vi "VI control.vi"() -> ()   [LabVIEW 2021]
uses:
  <vilib>/DAQmx/read.llb/DAQmx Read (Counter DBL 1Chan 1Samp).vi
  <vilib>/DAQmx/write.llb/DAQmx Write (Analog DBL 1Chan 1Samp).vi
  <vilib>/DAQmx/write.llb/DAQmx Write (Digital 1D Bool 1Chan 1Samp).vi
  <vilib>/DAQmx/create/channels.llb/DAQmx Create Channel (CI-Position-Angular Encoder).vi
  <vilib>/DAQmx/create/channels.llb/DAQmx Create Channel (AO-Voltage-Basic).vi
  <vilib>/DAQmx/create/channels.llb/DAQmx Create Channel (DO-Digital Output).vi
  <vilib>/DAQmx/miscellaneous.llb/DAQmx Fill In Error Info.vi
  <resource>/objmgr/daqmx.rc
panel:
  out "error out":errorcluster
  in  "umin":dbl=0.02
  out "Velocidad angular [°/s]":dbl(graph)
  in  "AOmax":dbl=5.0
  in  "AO02":dbl=0.2
  in  "AO01":dbl=0.2
  in  "rT2":dbl=0.99
  in  "rT1":dbl=0.94
  in  "lines":tag="Dev1/port0/line2, Dev1/port0/line1"
  in  "counter":tag="Dev1/ctr0"
  in  "physical channels":tag="Dev1/ao0"
  out "AO [V]":dbl
  out "Estado":dbl
  out "Señal de Control u":dbl(graph)
  out "Error []":dbl(graph)
  out "Angulo [°]":dbl(graph)
  in  "Stop":bool
  in  "tauM":dbl=0.1
  in  "zeta":dbl=0.08
  in  "Th0":dbl=2.0
  in  "wn":dbl=4.7
  in  "Nv":dbl
  in  "Limite":dbl=17.0
  in  "Kd":dbl=0.03
  in  "Ventana":dbl=3.0
  in  "Ki":dbl=0.02
  in  "Sentido":dbl=-1.0
  in  "Kp":dbl=0.03
  in  "Compensación":bool=TRUE
  in  "Simular":bool
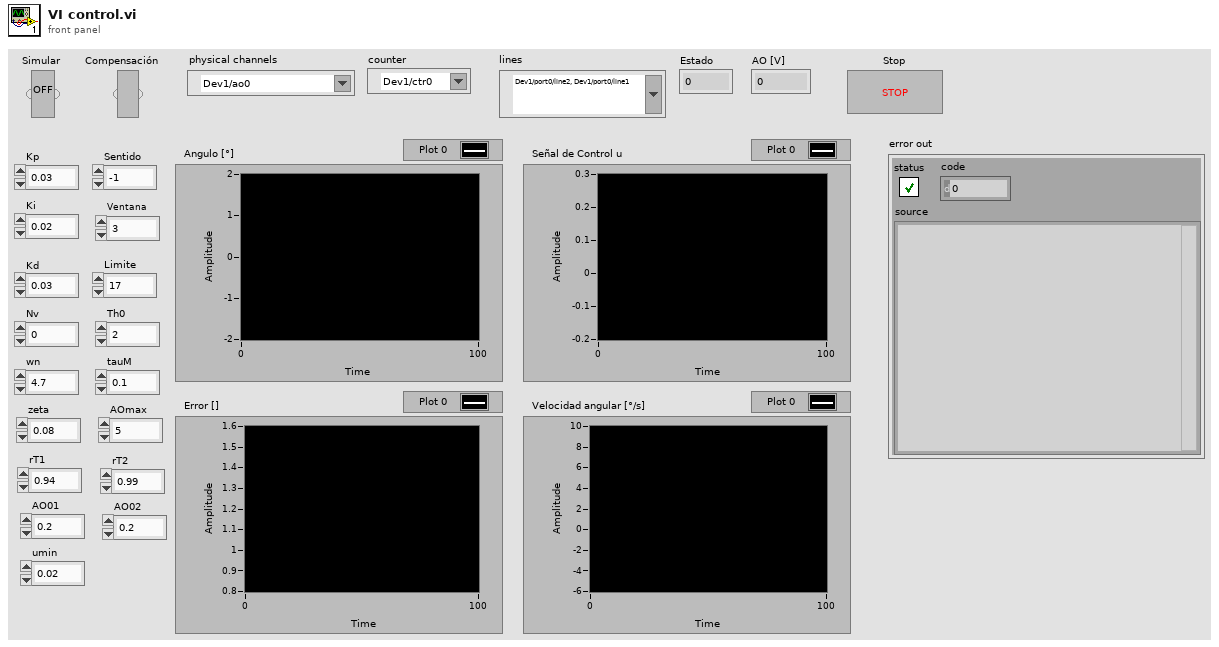
[diagram p1: front panel]
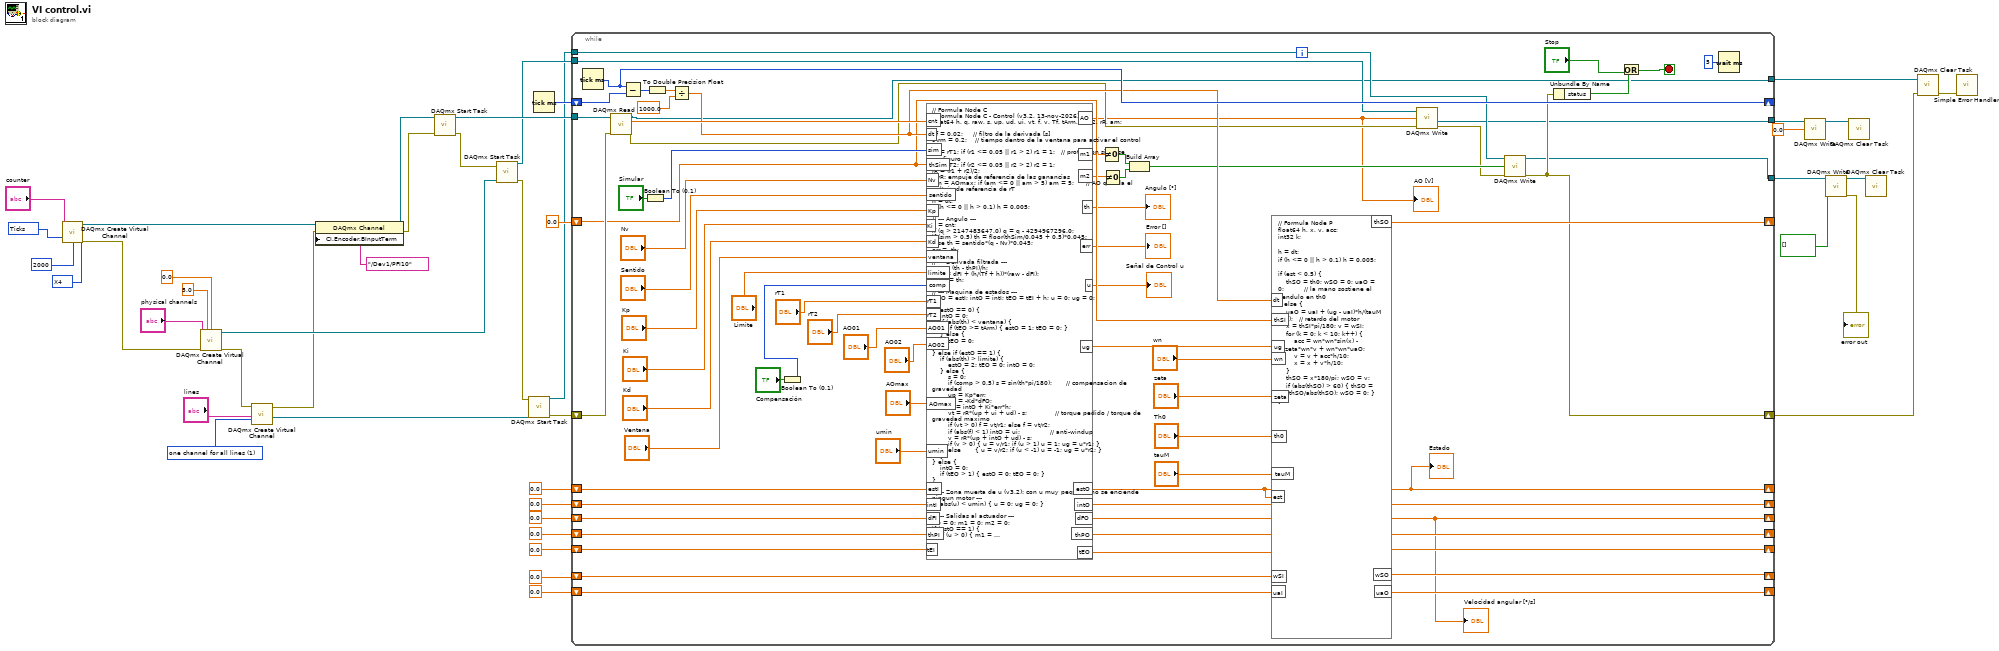
[diagram p0: block diagram]
diagram:
  w36 = 1 items=["one channel for each line", "one channel for all lines"] ("line grouping")
  w33 = 10304 items=["Degrees"=10146, "Radians"=10273, "Ticks"=10304, "From Custom Scale"=10065] ("units")
  w43 = 10092 items=["X1"=10090, "X2"=10091, "X4"=10092, "Two Pulse Counting"=10313] ("decoding type")
  n1 = call-poly <vilib>:"DAQmx Create Virtual Channel.vi"("counter"="counter", "decoding type"=w43, "units"=w33, "pulses per revolution"=u32 2000) -> ("task out"=w31:refnum<k21>, "error out"=w28:errorcluster)  [unwired: 10 in]
  n2 = call-poly <vilib>:"DAQmx Create Virtual Channel.vi"("maximum value"=5.0, "minimum value"=0.0, "physical channels"="physical channels", "error in"=w28) -> ("task out"=w35:refnum<k21>, "error out"=w27:errorcluster)  [unwired: 10 in]
  n3 = call-poly <vilib>:"DAQmx Create Virtual Channel.vi"("lines"="lines", "line grouping"=w36, "error in"=w27) -> ("task out"=w34:refnum<k21>, "error out"=w26:errorcluster)  [unwired: 11 in]
  n4 = property class="DAQmx Channel"(reference=w31, error in=w26, "CI.Encoder.BInputTerm"=tag "/Dev1/PFI10") -> (reference out=w30:refnum<k21>, error out=w29:errorcluster)
  n5 = call <vilib>:"DAQmx Start Task.vi"("task/channels in"=w30, "error in"=w29) -> ("task out"=w22:refnum<k21>, "error out"=w25:errorcluster)  [unwired: 12 in]
  n6 = call <vilib>:"DAQmx Start Task.vi"("task/channels in"=w35, "error in"=w25) -> ("task out"=w12:refnum<k21>, "error out"=w24:errorcluster)  [unwired: 12 in]
  n7 = call <vilib>:"DAQmx Start Task.vi"("task/channels in"=w34, "error in"=w24) -> ("task out"=w11:refnum<k21>, "error out"=w23:errorcluster)  [unwired: 12 in]
  n8 = Tick Count (ms)() -> (millisecond timer value=w21:u32)
  n9 = while {
    shift-right: [w105] -> _
    shift-left: w21 -> [w110]
    shift-right: [w73] -> _
    shift-left: 0.0 -> [w74]
    shift-right: [w70] -> _
    shift-left: 0.0 -> [w72]
    shift-right: [w69] -> _
    shift-left: 0.0 -> [w71]
    shift-right: [w83] -> _
    shift-left: 0.0 -> [w84]
    shift-right: [w56] -> _
    shift-left: 0.0 -> [w88]
    shift-right: [w82] -> _
    shift-left: 0.0 -> [w85]
    shift-right: [w81] -> _
    shift-left: 0.0 -> [w87]
    shift-right: [w48] -> _
    shift-left: 0.0 -> [w86]
    shift-right: [w53] -> w8
    shift-left: w23 -> [w104]
    tunnel: w22 -> [w111]
    tunnel: w12 -> [w61]
    tunnel: w11 -> [w62]
    tunnel: [w46] -> w4
    tunnel: [w45] -> w3
    tunnel: [w44] -> w2
    stop <- w50 stop-if-true
    n10 = Tick Count (ms)() -> (millisecond timer value=w105:u32)
    n11 = call-poly <vilib>:"DAQmx Read.vi"("task/channels in"=w111, "error in"=w104) -> ("task out"=w46:refnum<k21>, "data"=w109:dbl, "error out"=w68:errorcluster)  [unwired: 11 in]
    n12 = Subtract(x=w105, y=w110) -> (x-y=w108:u32)
    n13 = Boolean To (0,1)(Boolean="Simular") -> (0, 1=w102:i16)
    n14 = To Double Precision Float(number=w108) -> (double precision float=w107:dbl)
    n15 = Divide(x=w107, y=1000.0) -> (x/y=w79:dbl)
    n16 = Boolean To (0,1)(Boolean="Compensación") -> (0, 1=w100:i16)
    n17 = formula code="// Formula Node C\n// Formula Node C - Control (v3.2, 13-nov-2026)\nfloat64 h, q, raw, s, up, ud, ui, vt, f, v, Tf, tArm, r1, r2, rR, am;\n\nTf = 0.02;     // filtro de la derivada [s]\ntArm = 0.2;    // tiempo dentro de la ventana para activar el control [s]\nr1 = rT1; if (r1 <= 0.05 || r1 > 2) r1 = 1;   // proteccion si no se configuro\nr2 = rT2; if (r2 <= 0.05 || r2 > 2) r2 = 1;\nrR = (r1 + r2)/2;\n// rR: empuje de referencia de las ganancias\nam = AOmax; if (am <= 0 || am > 5) am = 5;      // AO que da el voltaje de referencia de rT\n\nh = dt;\nif (h <= 0 || h > 0.1) h = 0.005;\n\n// --- Angulo ---\nq = cnt;\nif (q > 2147483647.0) q = q - 4294967296.0;\nif (sim > 0.5) th = floor(thSim/0.045 + 0.5)*0.045;\nelse th = sentido*(q - Nv)*0.045;\nerr = -th;\n\n// --- Derivada filtrada ---\nraw = (th - thPI)/h;\ndFO = dFI + (h/(Tf + h))*(raw - dFI);\nthPO = th;\n\n// --- Maquina de estados ---\nestO = estI; intO = intI; tEO = tEI + h; u = 0; ug = 0;\n\nif (estO == 0) {\n    intO = 0;\n    if (abs(th) < ventana) {\n        if (tEO >= tArm) { estO = 1; tEO = 0; }\n    } else {\n        tEO = 0;\n    }\n} else if (estO == 1) {\n    if (abs(th) > limite) {\n        estO = 2; tEO = 0; intO = 0;\n    } else {\n        s = 0;\n        if (comp > 0.5) s = sin(th*pi/180);       // compensacion de gravedad\n        up = Kp*err;\n        ud = -Kd*dFO;\n        ui = intO + Ki*err*h;\n        vt = rR*(up + ui + ud) - s;              // torque pedido / torque de gravedad maximo\n        if (vt > 0) f = vt/r1; else f = vt/r2;\n        if (abs(f) < 1) intO = ui;               // anti-windup\n        v = rR*(up + intO + ud) - s;\n        if (v > 0) { u = v/r1; if (u > 1) u = 1; ug = u*r1; }\n        else       { u = v/r2; if (u < -1) u = -1; ug = u*r2; }\n    }\n} else {\n    intO = 0;\n    if (tEO > 1) { estO = 0; tEO = 0; }\n}\n\n// --- Zona muerta de u (v3.2): con u muy pequeno no se enciende ningun motor ---\nif (abs(u) < umin) { u = 0; ug = 0; }\n\n// --- Salidas al actuador ---\nAO = 0; m1 = 0; m2 = 0;\nif (estO == 1) {\n    if (u > 0) { m1 = 1; AO = AO01 + (am - AO01)*sqrt(u); }\n    if (u < 0) { m2 = 1; AO = AO02 + (am - AO02)*sqrt(-u); }\n}"("cnt"=w109, "dt"=w79, "sim"=w102, "thSim"=w74, "Nv"="Nv", "sentido"="Sentido", "Kp"="Kp", "Ki"="Ki", "Kd"="Kd", "ventana"="Ventana", "limite"="Limite", "comp"=w100, "rT1"="rT1", "rT2"="rT2", "AO01"="AO01", "AO02"="AO02", "estI"=w88, "intI"=w87, "dFI"=w86, "thPI"=w85, "tEI"=w84, "AOmax"="AOmax", "umin"="umin") -> ("th"=→"Angulo [°]":dbl, "err"=→"Error []":dbl, "u"=→"Señal de Control u":dbl, "ug"=w80:dbl, "AO"=w55:dbl, "m1"=w67:dbl, "m2"=w66:dbl, "estO"=w56:dbl, "intO"=w81:dbl, "dFO"=w48:dbl, "thPO"=w82:dbl, "tEO"=w83:dbl)
    "Estado" <- w56
    "AO [V]" <- w55
    "Velocidad angular [°/s]" <- w48
    n18 = Not Equal To 0?(x=w67) -> (x != 0?=w65:bool)
    n19 = Not Equal To 0?(x=w66) -> (x != 0?=w64:bool)
    n20 = Build Array(w65, w64) -> (w63:bool[])
    n21 = formula code="// Formula Node P\nfloat64 h, x, v, acc;\nint32 k;\n\nh = dt;\nif (h <= 0 || h > 0.1) h = 0.005;\n\nif (est < 0.5) {\n    thSO = th0; wSO = 0; uaO = 0;          // la mano sostiene el pendulo en th0\n} else {\n    uaO = uaI + (ug - uaI)*h/(tauM + h);   // retardo del motor\n    x = thSI*pi/180; v = wSI;\n    for (k = 0; k < 10; k++) {\n        acc = wn*wn*sin(x) - 2*zeta*wn*v + wn*wn*uaO;\n        v = v + acc*h/10;\n        x = x + v*h/10;\n    }\n    thSO = x*180/pi; wSO = v;\n    if (abs(thSO) > 60) { thSO = 60*thSO/abs(thSO); wSO = 0; }\n}"("est"=w56, "dt"=w79, "wn"="wn", "zeta"="zeta", "th0"="Th0", "tauM"="tauM", "thSI"=w74, "wSI"=w72, "uaI"=w71, "ug"=w80) -> ("thSO"=w73:dbl, "wSO"=w70:dbl, "uaO"=w69:dbl)
    n22 = call-poly <vilib>:"DAQmx Write.vi"("task/channels in"=w61, "data"=w55, "error in"=w68) -> ("task out"=w45:refnum<k21>, "error out"=w60:errorcluster)  [unwired: 10 in, 1 out]
    n23 = call-poly <vilib>:"DAQmx Write.vi"("task/channels in"=w62, "data"=w63, "error in"=w60) -> ("task out"=w44:refnum<k21>, "error out"=w53:errorcluster)  [unwired: 10 in, 1 out]
    n24 = Unbundle By Name(w53) -> ("status"=w52:bool)
    n25 = Or(x=w52, y="Stop") -> (x .or. y?=w50:bool)
    n26 = Wait (ms)(milliseconds to wait=u32 5) -> ()  [unwired: 1 out]
  }
  n27 = call-poly <vilib>:"DAQmx Write.vi"("task/channels in"=w3, "data"=0.0) -> ("task out"=w7:refnum<k21>)  [unwired: 11 in, 2 out]
  n28 = call-poly <vilib>:"DAQmx Write.vi"("task/channels in"=w2, "data"=bool[] []) -> ("task out"=w6:refnum<k21>, "error out"=→"error out":errorcluster)  [unwired: 11 in, 1 out]
  n29 = call <vilib>:"DAQmx Clear Task.vi"("task in"=w7) -> ()  [unwired: 14 in, 1 out]
  n30 = call <vilib>:"DAQmx Clear Task.vi"("task in"=w6) -> ()  [unwired: 14 in, 1 out]
  n31 = call <vilib>:"DAQmx Clear Task.vi"("task in"=w4, "error in"=w8) -> ("error out"=w5:errorcluster)  [unwired: 13 in]
  n32 = call <vilib>:"Simple Error Handler.vi"("error in (no error)"=w5) -> ()  [unwired: 4 in, 5 out]
